vi "Split Text into Words.vi"(8 "error in (no error)":errorcluster) -> (0 "error out":errorcluster)   [LabVIEW 2021, in "Text-Based VI Icon Unit Tests.lvlib"]
doc: "Contains all the tests related to the function Split Text to Words"
uses:
  Text-Based VI Icon Unit Tests.lvlib
  <vilib>/addons/_JKI Toolkits/Caraya/classes/Assert/Assert Equal Value_Variant.vi
  <vilib>/LabVIEW Icon API/Set Text Icon/Text-Based VI Icon.lvlib
  <vilib>/addons/_JKI Toolkits/Caraya/classes/Test/Test.lvclass
  <vilib>/addons/_JKI Toolkits/Caraya/classes/Assert/Assert.lvclass
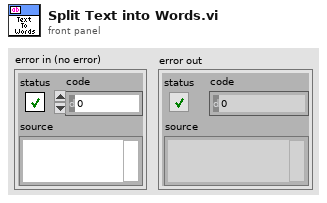
[diagram p1: front panel]
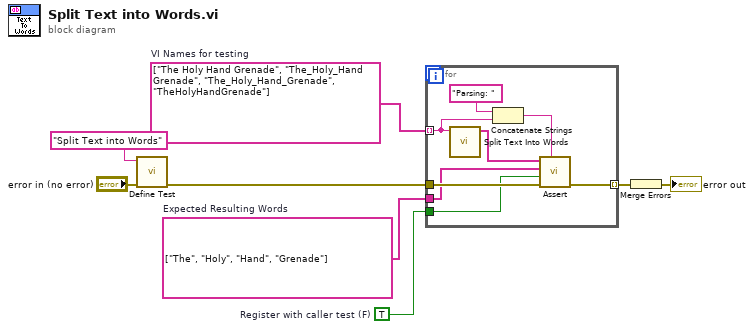
[diagram p0: block diagram]
diagram:
  w2 = TRUE  # Register with caller test (F)
  w6 = string[] ["The", "Holy", "Hand", "Grenade"]  # Expected Resulting Words
  w8 = string[] ["The Holy Hand Grenade", "The_Holy_Hand Grenade", "The_Holy_Hand_Grenade", "TheHolyHandGrenade"]  # VI Names for testing
  n1 = call <vilib>:"Define Test.vi"("error in (no error)"="error in (no error)", "Label (VI Title)"="Split Text into Words") -> ("error out"=w7:errorcluster)  [unwired: 8 in, 1 out]
  n2 = for {
    tunnel: w8 -> [w12] mode=indexing
    tunnel: w7 -> [w16]
    tunnel: [w15] -> w5 mode=indexing
    tunnel: w6 -> [w14]
    tunnel: w2 -> [w9]
    n3 = call <vilib>:"Split Text Into Words.vi"("VI Name"=w12) -> ("Array"=w13:string[])  [unwired: 10 in]
    n4 = Concatenate Strings("Parsing: ", w12) -> (w10:string)
    n5 = call-poly <vilib>:"Assert.vi"("Label"=w10, "error in (no error)"=w16, "Register with caller test (F)"=w9, "Y"=w14, "X"=w13) -> ("error out"=w15:errorcluster)  [unwired: 5 in, 1 out]
  }
  n6 = Merge Errors(w5) -> (→"error out":errorcluster)
